vi "Get U64.vi"(8 "error in (no error)":errorcluster, 10 "Name":string, 11 "json class in":refnum<class "json class.lvclass">) -> (0 "error out":errorcluster, 2 "U64":u64, 3 "json class out":refnum<class "json class.lvclass">)   [LabVIEW 2021, in "Config Library.lvlib" / "json class.lvclass"]
uses:
  json class.lvclass
  json class.lvclass/json class.ctl
  <vilib>/addons/JSON API/JSON Value/JSON Value.lvclass
  <vilib>/addons/JSON API/JSON Scalar/JSON Scalar.lvclass
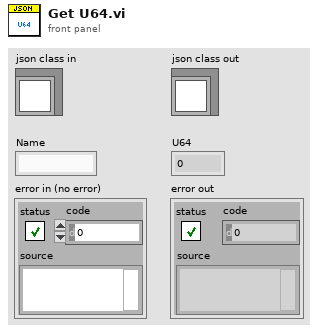
[diagram p1: front panel]
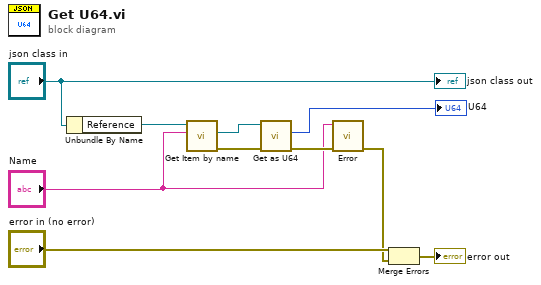
[diagram p0: block diagram]
diagram:
  n1 = Unbundle By Name("json class in") -> ("Reference"=w8:refnum<class "JSON Value.lvclass">)
  n2 = call-dynamic "Get Item by name.vi"("name"="Name", "JSON Value In"=w8) -> ("error out"=w4:errorcluster, "Value"=w7:refnum<class "JSON Value.lvclass">)  [unwired: 6 in, 2 out]
  n3 = call <vilib>:"Get as U64.vi"("error in (no error)"=w4, "JSON Scalar in"=w7) -> ("error out"=w3:errorcluster, "Number"=→"U64":u64)  [unwired: 7 in, 1 out]
  n4 = call "Error.vi"("error in (no error)"=w3, "Name"="Name") -> ("error out"=w1:errorcluster)  [unwired: 9 in]
  n5 = Merge Errors("error in (no error)", w1) -> (→"error out":errorcluster)
  "json class out" <- "json class in"
